vi "Release Object Reference.vi"(8 "error in":errorcluster, 11 "object":T1) -> (0 "error out":errorcluster)   [LabVIEW 2026, in "ToastNotification.lvlib" / "Reflection DotNet.lvlib"]
doc: "Close one acquired .NET reference if valid, including with an incoming error. Null and already closed handles require no action. Preserve the incoming error and merge cleanup failures. Does not invoke IDisposable.Dispose. Never use this helper to close borrowed callback arguments or reference-out aliases as separate acquisitions."
uses:
  Reflection DotNet.lvlib
  Callback Object Reference.ctl
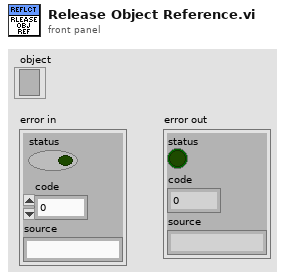
[diagram p1: front panel]
types:
  T1 = typedef "ToastNotification.lvlib/Reflection DotNet.lvlib/Callback Object Reference.ctl" = refnum<k24>
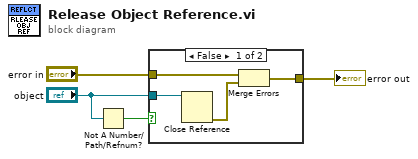
[diagram p0: block diagram]
diagram:
  n1 = Not A Number/Path/Refnum?(number/path/refnum="object") -> (NaN/Path/Refnum?=w3:bool)
  n2 = case shown="False" w3 {
    tunnel: "object" -> [w5 _]
    tunnel: "error in" -> [w6 w9]
    tunnel: [w8 w9] -> w4
    frame False {
      n3 = Close Reference(reference=w5) -> (error out=w7:errorcluster)  [unwired: 1 in]
      n4 = Merge Errors(w6, w7) -> (w8:errorcluster)
    }
    frame True {
    }
  }
  "error out" <- w4
